vi "List Topic Subscriptions Recursive.vi"(8 "error in (no error)":errorcluster, 10 "NextToken":string, 11 "Topic":refnum<class "Topic.lvclass">) -> (0 "error out":errorcluster, 3 "Topic Subscriptions":refnum<class "Subscription.lvclass">[](array[class]))   [LabVIEW 2015, in "NI_AWS_SNS.lvlib" / "Topic.lvclass"]
uses:
  Topic.lvclass
  Subscription/Subscription.lvclass
  Core/HTTP Request/Request Options.ctl
  Core/HTTP Request/Name Value Pair.ctl
  Core/HTTP Request/Region handling.ctl
  Core/HTTP Request/URL formatting.ctl
  Core/ARN/ARN.lvclass/ARN.ctl
  Core/HTTP Request/HTTP Request.lvclass/HTTP Request.ctl
  Core/ARN/Read ARN.vi
  Core/HTTP Request/Read Credentials.vi
  Core/HTTP Request/Read Service.vi
  Core/HTTP Request/Read Verify Server.vi
  Core/HTTP Request/Write Credentials.vi
  Core/HTTP Request/Write Region.vi
  Core/HTTP Request/Write Service.vi
  Core/HTTP Request/Write Verify Server.vi
  Core/HTTP Request/HTTP Request.lvclass
  XML Parsing/NI_XML Parsing.lvlib
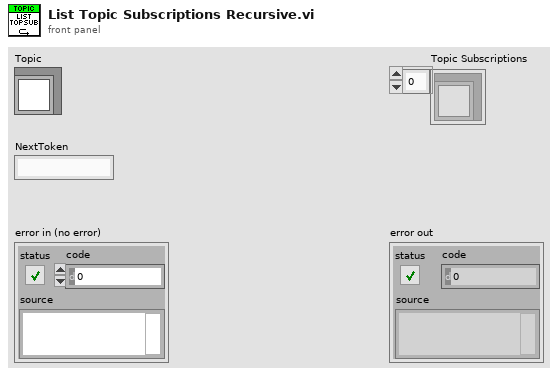
[diagram p1: front panel]
types:
  T1 = typedef "NI_AWS_Core.lvlib/HTTP Request.lvclass/Name Value Pair.ctl" = cluster{"name":string, "value":string}
  T2 = typedef "NI_AWS_Core.lvlib/HTTP Request.lvclass/Request Options.ctl" = cluster{"request headers":T1[], "request parameters":T1[], "request body":string, "region handling":T3, "URL formatting":T4}
  T3 = typedef "NI_AWS_Core.lvlib/HTTP Request.lvclass/Region handling.ctl" = enum16{"use region everywhere", "use region (authentication only)", "use region (URL only)", "ignore region everwhere"}
  T4 = typedef "NI_AWS_Core.lvlib/HTTP Request.lvclass/URL formatting.ctl" = enum16{"region-", "region."}
  T5 = typedef "NI_AWS_Core.lvlib/HTTP Request.lvclass/Response.ctl" = cluster{"Headers":string, "Body":string}
  T6 = typedef "NI_AWS_Core.lvlib/HTTP Request.lvclass/AWS Credentials.ctl" = cluster{"Access Key":string, "Secret Key":string}
  T7 = typedef "NI_AWS_Core.lvlib/HTTP Request.lvclass/Region.ctl" = enum16{"us-east-1", "us-east-2", "us-west-1", "us-west-2", "ap-northeast-1", "ap-northeast-2", "ap-southeast-1", "ap-southeast-2", "ca-central-1", "eu-central-1", "eu-west-1", "eu-west-2", "sa-east-1"}
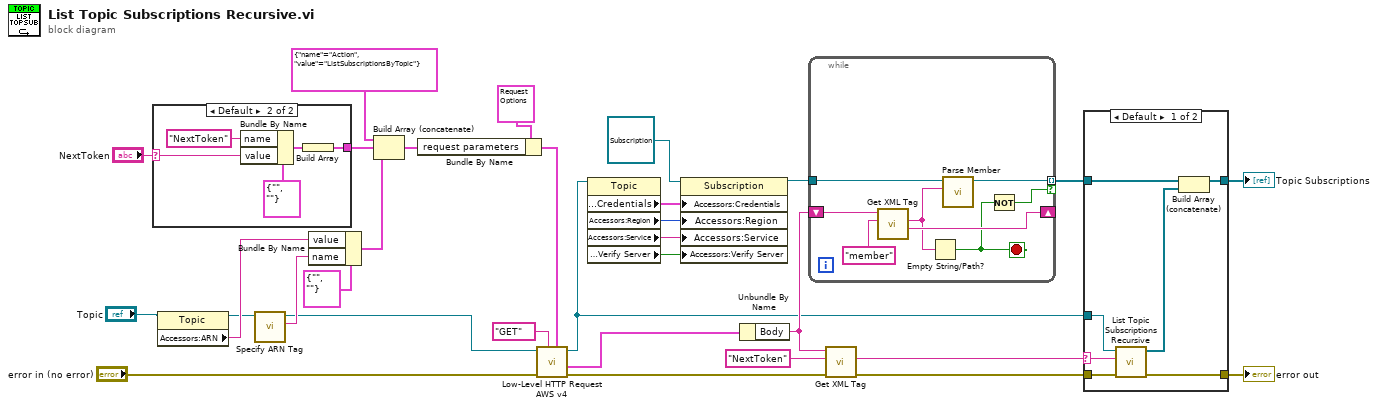
[diagram p0: block diagram]
diagram:
  n1 = case shown="Default" "NextToken" {
    selector: "NextToken" -> [_ w36]
    tunnel: [_ w32] -> w30
    frame "" {
    }
    frame Default {
      n2 = Bundle By Name(cluster=T1 {"name"="", "value"=""} ("Name Value Pair"), "name"="NextToken", "value"=w36) -> (w34:T1)
      n3 = Build Array(w34) -> (w32:T1[])
    }
  }
  n4 = property class="Topic"(reference="Topic") -> (reference out=w17:refnum<class "Topic.lvclass">, "Accessors:ARN"=w18:string)  [unwired: 1 in, 1 out]
  n5 = call-dynamic "Specify ARN Tag.vi"("Topic in"=w17) -> ("ARN Tag"=w14:string, "Topic out"=w2:refnum<class "Topic.lvclass">)  [unwired: 9 in]
  n6 = Bundle By Name(cluster=T1 {"name"="", "value"=""} ("element"), "value"=w18, "name"=w14) -> (w15:T1)
  n7 = Build Array (concatenate)(T1 {"name"="Action", "value"="ListSubscriptionsByTopic"} ("Name Value Pair"), w30, w15) -> (w28:T1[])
  n8 = Bundle By Name(cluster=T2 {"request headers"=[], "request parameters"=[{"name"="Action", "value"="ListQueues"}], "request body"="", "region handling"=enum."use region everywhere", "URL formatting"=enum."region."} ("Request Options"), "request parameters"=w28) -> (w3:T2)
  n9 = call "Low-Level HTTP Request AWS v4.vi"("Request Options"=w3, "HTTP-Verb"="GET", "error in (no error)"="error in (no error)", "AWS Core in"=w2) -> ("error out"=w21:errorcluster, "Response"=w5:T5, "AWS Core out"=w1:refnum<class "Topic.lvclass">)  [unwired: 4 in, 1 out]
  n10 = property class="Topic"(reference=w1) -> ("Accessors:Credentials"=w9:T6, "Accessors:Region"=w8:T7, "Accessors:Service"=w7:string, "Accessors:Verify Server"=w6:bool)  [unwired: 1 in, 2 out]
  n11 = property class="Subscription"(reference=refnum<class "Subscription.lvclass"> refnum ("NI_AWS_SNS.lvlib:Subscription"), "Accessors:Credentials"=w9, "Accessors:Region"=w8, "Accessors:Service"=w7, "Accessors:Verify Server"=w6) -> (reference out=w10:refnum<class "Subscription.lvclass">)  [unwired: 1 in, 1 out]
  n12 = Unbundle By Name(w5) -> ("Body"=w13:string)
  n13 = while {
    shift-right: [w42] -> _
    shift-left: w13 -> [w44]
    tunnel: [w41] -> w12 mode=indexing if=w38
    tunnel: w10 -> [w37]
    stop <- w39 stop-if-true
    n14 = call "Get XML Tag.vi"("Tag name"="member", "XML String in"=w44) -> ("Remaining string"=w42:string, "Tag value"=w40:string)  [unwired: 5 in, 3 out]
    n15 = Empty String/Path?(string/path=w40) -> (empty?=w39:bool)
    n16 = call-dynamic "Parse Member.vi"("member"=w40, "Subscription in"=w37) -> ("Subscription out"=w41:refnum<class "Subscription.lvclass">)  [unwired: 8 in, 1 out]
    n17 = Not(x=w39) -> (.not. x?=w38:bool)
  }
  n18 = call "Get XML Tag.vi"("error in (no error)"=w21, "Tag name"="NextToken", "XML String in"=w13) -> ("error out"=w20:errorcluster, "Tag value"=w24:string)  [unwired: 4 in, 3 out]
  n19 = case shown="Default" w24 {
    selector: w24 -> [w47 _]
    tunnel: w12 -> [w51 w53]
    tunnel: [w50 w53] -> w23
    tunnel: w20 -> [w49 w52]
    tunnel: [w48 w52] -> w22
    tunnel: w1 -> [w46 _]
    frame Default {
      n20 = call "List Topic Subscriptions Recursive.vi"("error in (no error)"=w49, "NextToken"=w47, "Topic"=w46) -> ("error out"=w48:errorcluster, "Topic Subscriptions"=w45:refnum<class "Subscription.lvclass">[])  [unwired: 7 in]
      n21 = Build Array (concatenate)(w51, w45) -> (w50:refnum<class "Subscription.lvclass">[])
    }
    frame "" {
    }
  }
  "error out" <- w22
  "Topic Subscriptions" <- w23
